vi "Create String Control for Path.vi"(0 "VI Refnum":refnum<vi>, 1 "Typedef Cluster":refnum<vi>, 5 "Path Refnum":refnum<vi>, 11 "error in (no error)":errorcluster) -> (4 "Reference String":string, 6 "String ctl ref":refnum<vi>, 15 "error out":errorcluster)   [LabVIEW 2021, in "Migrator.lvlib"]
uses:
  Migrator.lvlib
  <vilib>/Utility/miscctls.llb/LVPositionTypeDef.ctl
  <vilib>/Utility/miscctls.llb/LVPointTypeDef.ctl
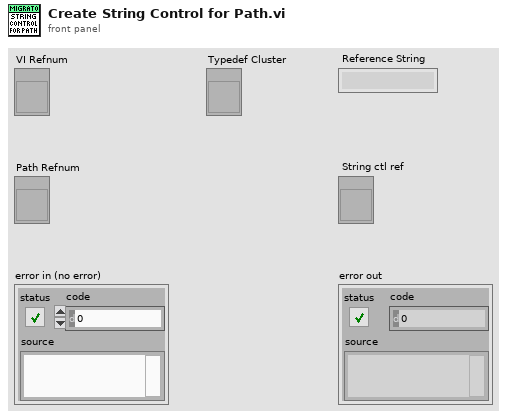
[diagram p1: front panel]
types:
  T1 = typedef "LVPointTypeDef.ctl" = cluster{"Horizontal":i16, "Vertical":i16}
  T2 = typedef "LVPositionTypeDef.ctl" = cluster{"Left":i32, "Top":i32}
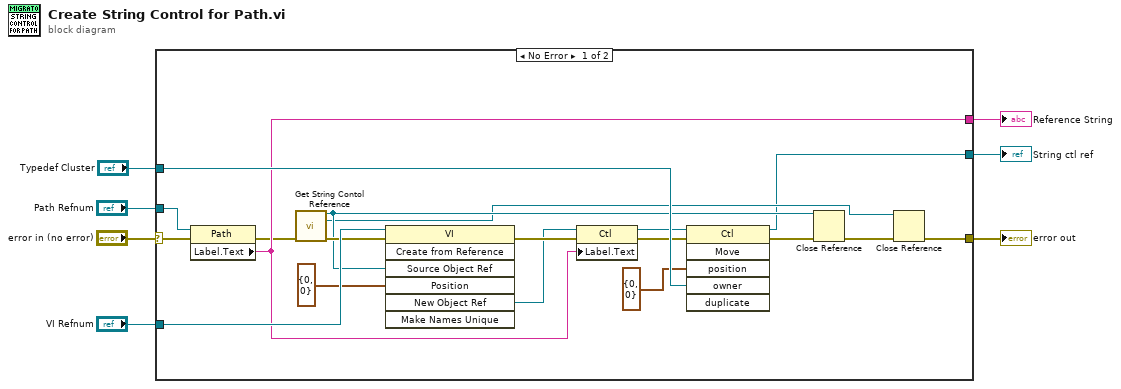
[diagram p0: block diagram]
diagram:
  n1 = case shown="No Error" "error in (no error)" {
    selector: "error in (no error)" -> [w20 w27]
    tunnel: [w26 w27] -> w7
    tunnel: "Typedef Cluster" -> [w25 _]
    tunnel: "VI Refnum" -> [w24 _]
    tunnel: [w23 _] -> w4
    tunnel: "Path Refnum" -> [w21 _]
    tunnel: [w8 _] -> w1
    frame No Error {
      n2 = property class="Path"(reference=w21, error in=w20) -> (error out=w22:errorcluster, "Label.Text"=w23:string)  [unwired: 1 out]
      n3 = call "Get String Contol Reference.vi"("error in (no error)"=w22) -> ("String"=w17:refnum<vi>, "vi reference"=w10:refnum<vi>, "error out"=w19:errorcluster)  [unwired: 12 in]
      n4 = invoke class="VI" method="Create from Reference"(reference=w24, error in=w19, "Source Object Ref"=w17, "Position"=T1 {"Horizontal"=0, "Vertical"=0}) -> (error out=w16:errorcluster, "New Object Ref"=w15:refnum<vi>)  [unwired: 3 in, 5 out]
      n5 = property class="Ctl"(reference=w15, error in=w16, "Label.Text"=w23) -> (reference out=w14:refnum<vi>, error out=w13:errorcluster)
      n6 = invoke class="Ctl" method="Move"(reference=w14, error in=w13, "position"=T2 {"Left"=0, "Top"=0}, "owner"=w25) -> (reference out=w8:refnum<vi>, error out=w12:errorcluster)  [unwired: 2 in, 4 out]
      n7 = Close Reference(reference=w17, error in (no error)=w12) -> (error out=w9:errorcluster)
      n8 = Close Reference(reference=w10, error in (no error)=w9) -> (error out=w26:errorcluster)
    }
    frame Error {
    }
  }
  "error out" <- w7
  "Reference String" <- w4
  "String ctl ref" <- w1
